vi "Main.vi"(11 "Module Admin":refnum<class "Delacor_lib_QMH_Module Admin.lvclass">) -> ()   [LabVIEW 2020, in "Peek Window.lvlib"]
doc: "This template is based off of the Queued Message Handler design pattern and the Queued Message Handler project template that ships with LabVIEW.\n\nThe main difference is that the queue is private to this module and communication between modules is performed via Broadcast and Request events.\n\nRequest events are wrapped in public API methods and are handled in the Event Handling Loop (EHL) of this VI. Any module can register for Broadcast events sent by this module. The EHL generates messages based on user interface actions.\n\nThe Message Handling Loop (MHL) processes messages generated by the EHL, or by other messages. The messages are string values, so new messages can be added easily to the Message Cases case structure in the MHL. Each message cluster can also provide an optional value for Message Data, which is a variant that can be converted to whatever message-specific data is required.\n_____\nBased on Delacor QMH Project Template 5.0.0.82."
uses:
  Peek Window.lvlib
  <vilib>/Delacor/Delacor QMH/Libraries/Module Admin_class/Delacor_lib_QMH_Module Admin.lvclass
  MHL Data Cluster.ctl
  VI Types/Standard VI Type/Standard VI Type.lvclass
  EHL Data Cluster.ctl
  <vilib>/Delacor/Delacor QMH/Libraries/Message Queue_class/Delacor_lib_QMH_Message Queue.lvclass/Delacor_lib_QMH_Message Queue.ctl
  Stop Argument--cluster.ctl
  Open Diagram Argument--cluster.ctl
  Invalid Selection Argument--cluster.ctl
  VI Types/Standard VI Type/Standard VI Type.lvclass/Standard VI Type.ctl
  Scroll Data.ctl
  <vilib>/Utility/traverseref.llb/TRef TravTarget.ctl
  <vilib>/Delacor/Delacor QMH/Libraries/Module Admin_class/Delacor_lib_QMH_Module Admin.lvclass/Delacor_lib_QMH_Module Admin.ctl
  <vilib>/Delacor/Delacor QMH/Libraries/Message Queue_class/Delacor_lib_QMH_Enqueue Message (Single).vi
  VI Types/Standard VI Type/Read VI Refnum.vi
  VI Types/Standard VI Type/Read Full Qualified Name.vi
  <vilib>/Delacor/Delacor QMH/Libraries/Module Admin_class/Delacor_lib_QMH_Get External Launch.vi
  <vilib>/Utility/error.llb/Error Cluster From Error Code.vi
  <vilib>/ErrorRing/Error Ring.xnode
  <vilib>/Delacor/Delacor QMH/Libraries/Message Queue_class/Delacor_lib_QMH_Message Queue.lvclass
  <vilib>/Utility/miscctls.llb/LVPoint32TypeDef.ctl
panel:
  in  "File Open":bool
  in  "Previous":bool
  in  "Peek Stack":string(tree)
  out "Application":string
  in  "Simulate MHL Error":bool
  in  "Simulate EHL Error":bool
  out "error out":errorcluster
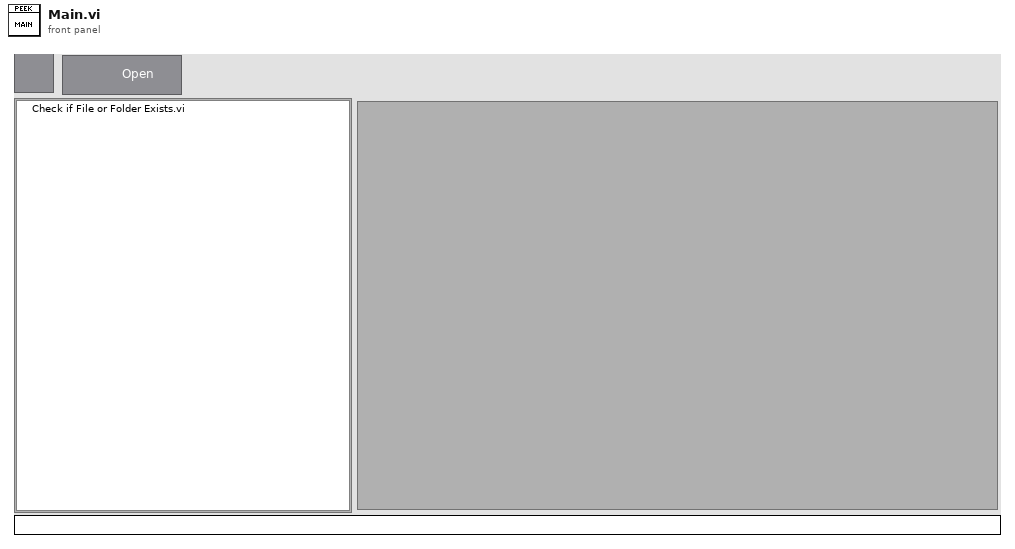
[diagram p1: front panel]
types:
  T1 = typedef "Peek Window.lvlib/EHL Data Cluster.ctl" = cluster{"VI Inserted":string, "Top VI":refnum<class "Standard VI Type.lvclass">}
  T2 = typedef "Peek Window.lvlib/MHL Data Cluster.ctl" = cluster{"PeekVI Reference":refnum<vi>, "SubPanel":refnum<vi>, "Peek Stack Tree Ref":refnum<vi>, "Open Button Ref":refnum<vi>, "Top VI":refnum<class "Standard VI Type.lvclass">, "Active VI":refnum<class "Standard VI Type.lvclass">, "Stack":refnum<class "Standard VI Type.lvclass">[], "Last FP State":enum32{"Invalid", "Standard", "Closed", "Hidden", "Minimized", "Maximized"}}
  T3 = typedef "Peek Window.lvlib/Request Events--cluster.ctl" = cluster{"Stop Module":refnum<user-event>, "Show Panel":refnum<user-event>, "Hide Panel":refnum<user-event>, "Get Module Execution Status":refnum<user-event>, "Show Diagram":refnum<user-event>, "Open Diagram":refnum<user-event>, "Invalid Selection":refnum<user-event>}
  T4 = enum32{"invalid lock state", "Not Locked", "Locked (No Password)", "Password-protected"}
  T5 = typedef "Peek Window.lvlib/Stop Argument--cluster.ctl" = cluster{"Origin":string, "Exit via Stop Module Req?":bool, "Wait for Module to stop?":bool}
  T6 = typedef "Peek Window.lvlib/Open Diagram Argument--cluster.ctl" = cluster{"VI Type":refnum<class "Standard VI Type.lvclass">}
  T7 = typedef "Peek Window.lvlib/Invalid Selection Argument--cluster.ctl" = cluster{"Active VI":string}
  T8 = enum32{"Invalid", "Standard", "Closed", "Hidden", "Minimized", "Maximized"}
  T9 = typedef "Peek Window.lvlib/Scroll Data.ctl" = cluster{"Coords":T10, "Delta":i32, "PlatMods":cluster{"Shift":bool, "Ctrl":bool, "Alt":bool, "Cmd":bool, "Opt":bool}}
  T10 = typedef "LVPoint32TypeDef.ctl" = cluster{"Horizontal":i32, "Vertical":i32}
  T11 = typedef "TRef TravTarget.ctl" = enum16{"FP", "BD", "Other"}
  T12 = cluster{"Shift":bool, "Ctrl":bool, "Alt":bool, "Cmd":bool, "Opt":bool}
  T13 = cluster{"Coords":T10, "Delta":i32, "PlatMods":cluster{"Shift":bool, "Ctrl":bool, "Alt":bool, "Cmd":bool, "Opt":bool}}
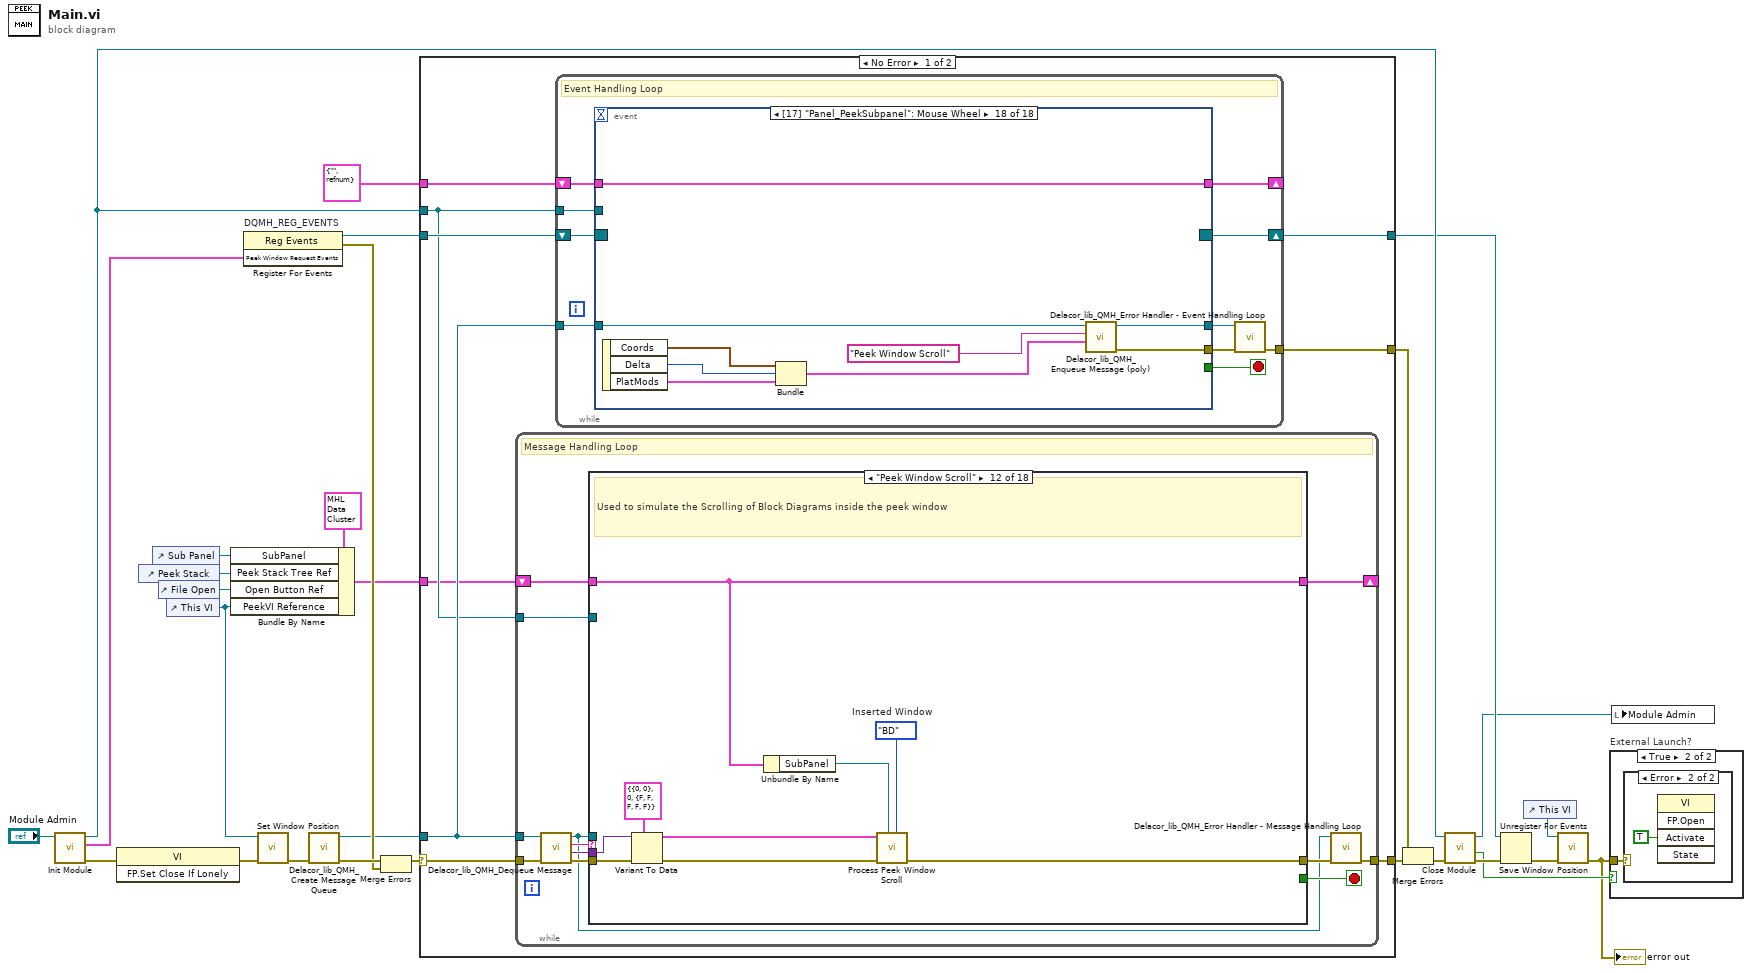
[diagram p0: block diagram]
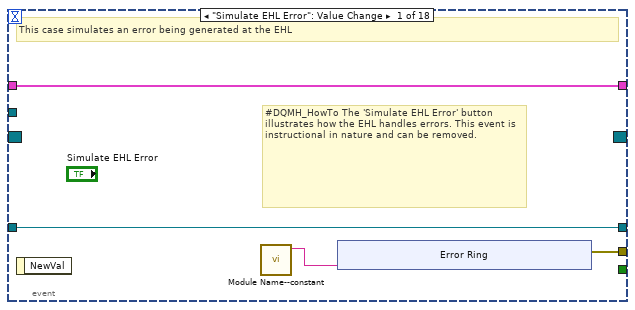
[diagram p2: hidden frame]
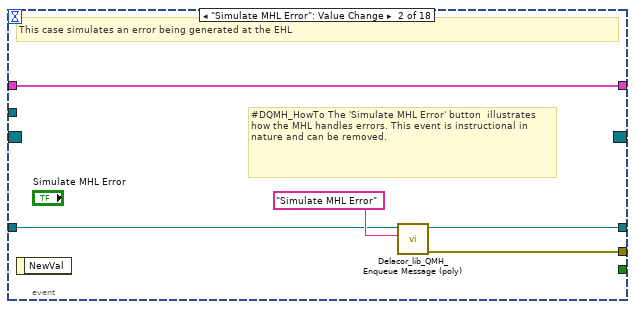
[diagram p3: hidden frame]
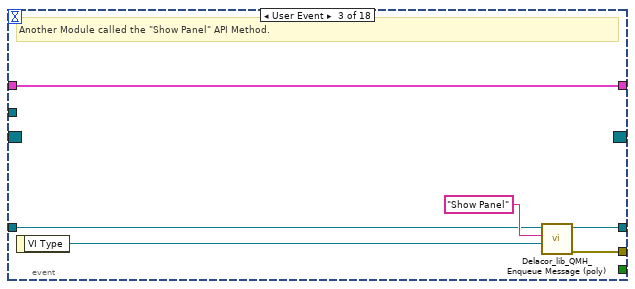
[diagram p4: hidden frame]
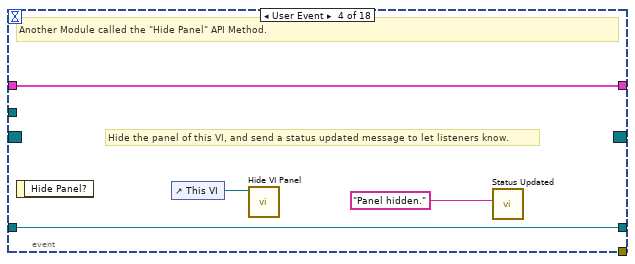
[diagram p5: hidden frame]
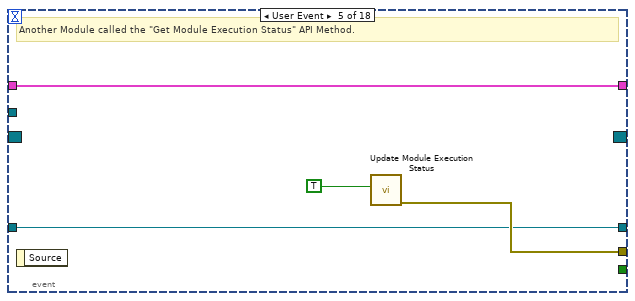
[diagram p6: hidden frame]
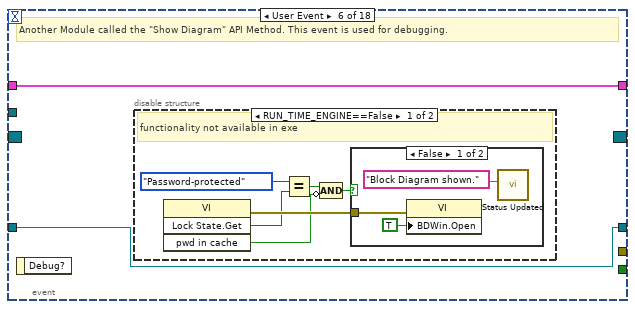
[diagram p7: hidden frame]
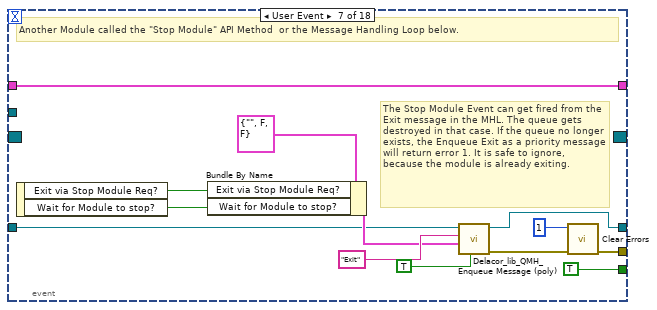
[diagram p10: hidden frame]
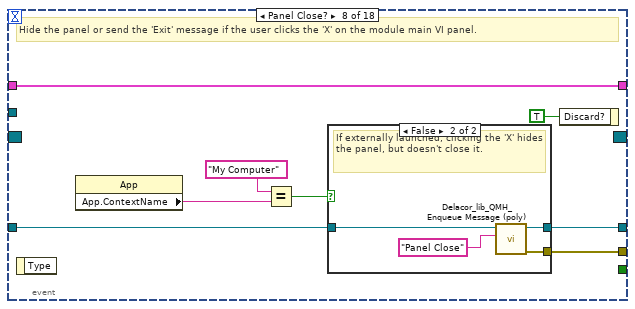
[diagram p11: hidden frame]
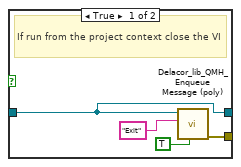
[diagram p12: hidden frame]
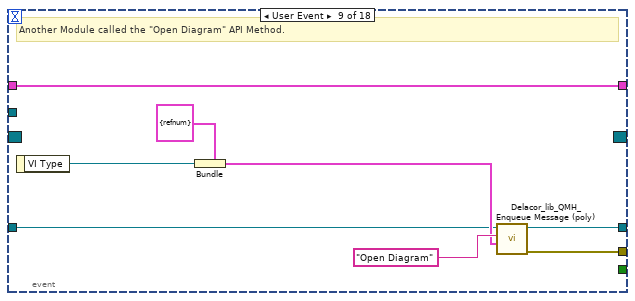
[diagram p13: hidden frame]
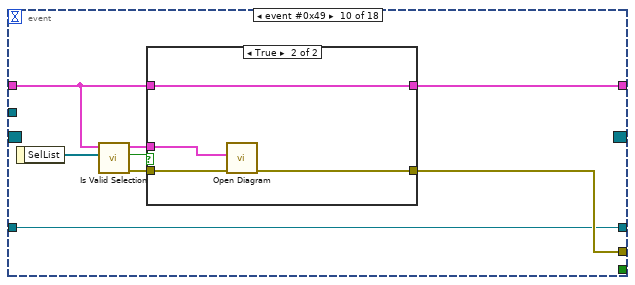
[diagram p14: hidden frame]
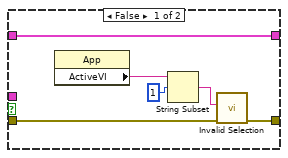
[diagram p15: hidden frame]
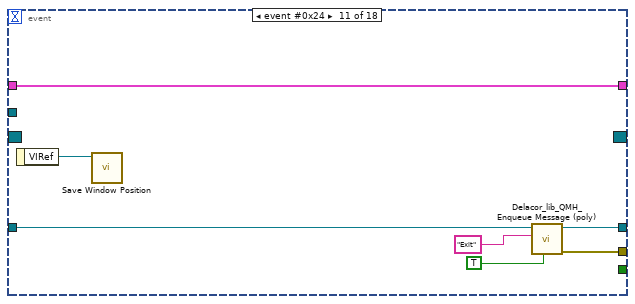
[diagram p16: hidden frame]
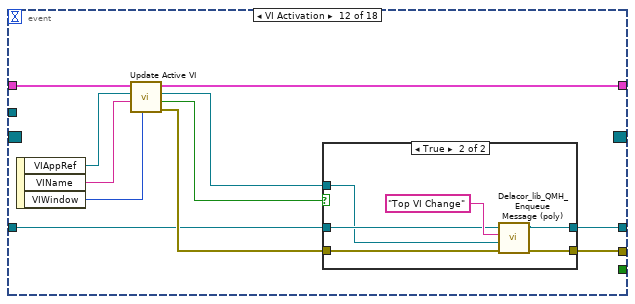
[diagram p17: hidden frame]
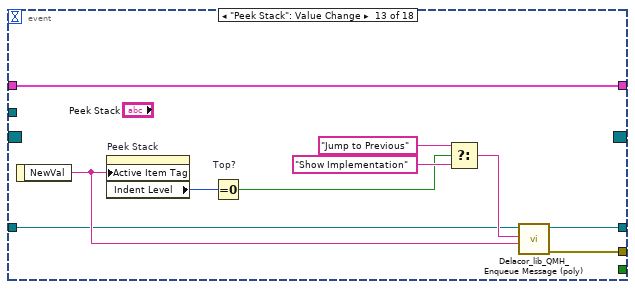
[diagram p19: hidden frame]
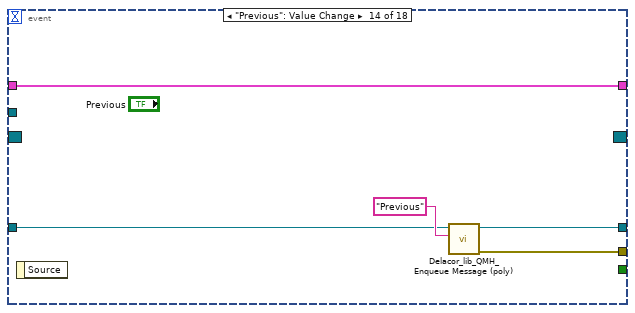
[diagram p20: hidden frame]
diagram:
  n1 = call "Init Module.vi"("Singleton Module Admin in"="Module Admin") -> ("error out"=w9:errorcluster, "Peek Window Request Events"=w18:T3, "Singleton Module Admin out"=w21:refnum<class "Delacor_lib_QMH_Module Admin.lvclass">)  [unwired: 8 in]
  n2 = invoke class="VI" method="FP.Set Close If Lonely"(error in=w9) -> (error out=w7:errorcluster)  [unwired: 2 in, 2 out]
  n3 = control-ref of="Peek Stack"() -> (w8:refnum<vi>)
  n4 = control-ref of="Sub Panel"() -> (w11:refnum<vi>)
  n5 = control-ref of="File Open"() -> (w1:refnum<vi>)
  n6 = control-ref of="This VI"() -> (w5:refnum<vi>)
  n7 = Bundle By Name(cluster=T2 {"PeekVI Reference"=refnum, "SubPanel"=refnum, "Peek Stack Tree Ref"=refnum, "Open Button Ref"=refnum, "Top VI"=refnum, "Active VI"=refnum, "Stack"=[], "Last FP State"=enum."Standard"} ("Data Cluster"), "SubPanel"=w11, "Peek Stack Tree Ref"=w8, "Open Button Ref"=w1, "PeekVI Reference"=w5) -> (w12:T2)
  n8 = register-events "DQMH_REG_EVENTS"(w18) -> (reference out=w19:refnum<event-registration>, error out=w22:errorcluster)  [unwired: 2 in]
  n9 = call "Set Window Position.vi"("error in"=w7, "VI Reference"=w5) -> ("error out"=w6:errorcluster)  [unwired: 9 in]
  n10 = call <vilib>:"Delacor_lib_QMH_Create Message Queue.vi"("error in"=w6) -> ("error out"=w24:errorcluster, "Message Queue"=w17:refnum<class "Delacor_lib_QMH_Message Queue.lvclass">)  [unwired: 9 in]
  n11 = Merge Errors(w24, w22) -> (w23:errorcluster)
  n12 = case shown="No Error" w23 {
    selector: w23 -> [w35 w498]
    tunnel: [w37 w497] -> w28
    tunnel: [w34 w503] -> w20
    tunnel: w19 -> [w33 w503]
    tunnel: w17 -> [w32 w496]
    tunnel: [w36 _] -> w26
    tunnel: w21 -> [w31 w499]
    tunnel: w12 -> [w30 _]
    tunnel: T1 {"VI Inserted"="", "Top VI"=refnum} ("Data") -> [w29 _]
    frame No Error {
      n13 = while {
        tunnel: w32 -> [w222]
        shift-right: [w219] -> _
        shift-left: w30 -> [w226]
        tunnel: w35 -> [w229]
        tunnel: [w227] -> w37
        tunnel: w31 -> [w220]
        stop <- w225 stop-if-true
        # "Message Handling Loop"
        n14 = call-dynamic "Delacor_lib_QMH_Dequeue Message.vi"("error in"=w229, "Message Queue in"=w222) -> ("error out"=w228:errorcluster, "Message Data"=w223:variant, "Message"=w224:string, "Message Queue out"=w221:refnum<class "Delacor_lib_QMH_Message Queue.lvclass">)  [unwired: 6 in]
        n15 = case "DQMH_MESSAGE_CASES" shown="\"Peek Window Scroll\"" w224 {
          selector: w224 -> [_ _ _ _ _ _ _ _ _ _ _ _ _ _ _ _ _ w483]
          tunnel: w221 -> [_ _ _ _ _ _ _ _ _ _ _ _ _ _ _ w453 w475 _]
          tunnel: w228 -> [w241 w243 w250 w265 w299 w316 w342 w354 w367 w384 w412 w432 w435 w437 w442 w460 w481 w485]
          tunnel: [w231 w243 w245 w262 w297 w319 w336 w351 w368 w383 w404 w427 w434 w437 w441 w456 w478 w486] -> w230
          tunnel: w226 -> [w235 w242 w246 w259 w293 w317 w333 w357 w363 w388 w400 w426 w433 w436 w439 w455 w474 w484]
          tunnel: [w232 w242 w247 w260 w296 w318 w334 w356 w361 w387 w399 w426 w433 w436 w439 w455 w474 w484] -> w219
          tunnel: [_ _ _ _ _ _ _ _ _ _ _ _ _ _ _ _ w473 _] -> w225
          tunnel: w223 -> [_ _ w249 w264 w298 _ w340 _ w365 _ w411 w430 _ _ _ w454 w472 _]
          tunnel: w220 -> [w238 _ _ _ _ _ _ _ _ _ _ _ _ _ _ w452 w467 _]
          frame "Initialize" {
            # "Initialize - Any operation that needs to be done before the module can receive messages. Synchronize Caller Events.vi will inform Start Module.vi that the module has launched and is ready to receive messages. Module Did Init.vi will broadcast that the module initialized."
            n16 = call "Synchronize Caller Events.vi"("error in (no error)"=w241, "Singleton Module Admin in"=w238) -> ("error out"=w240:errorcluster)  [unwired: 8 in, 1 out]
            n17 = call "Module Name--constant.vi"() -> ("Module Name"=w239:string)  [unwired: 11 in]
            n18 = property on="Property Node" class="VI"("Front Panel.Title"=w239) -> (reference out=w233:refnum<vi>)  [unwired: 2 in, 1 out]
            n19 = call "Initialize Tree.vi"("Module Data"=w235) -> ("Module Data"=w232:T2)  [unwired: 9 in, 1 out]
            n20 = call "Module Name--constant.vi"() -> ("Module Name"=w236:string)  [unwired: 11 in]
            n21 = property on="Property Node" class="VI"(reference=w233, "FP.State"=T8."Standard" ("Front Panel Window:State")) -> ()  [unwired: 1 in, 2 out]
            n22 = call "Module Did Init.vi"("error in (no error)"=w240, "Initialized?"=TRUE, "Origin"=w236) -> ("error out"=w231:errorcluster)  [unwired: 8 in]
          }
          frame "--- Module Specific ---" {
            # "Separator -- The following cases handle messages specific to this Module."
          }
          frame "Top VI Change" {
            w248 = refnum<class "Standard VI Type.lvclass"> refnum  # Top VI
            # "Open BD of selected SubVI"
            n23 = Variant To Data(error in=w250, type=w248, Variant=w249) -> (data=w244:refnum<class "Standard VI Type.lvclass">, error out=w245:errorcluster)
            n24 = Bundle By Name(cluster=w246, "Top VI"=w244) -> (w247:T2)
          }
          frame "Open Diagram" {
            # "Open BD of selected SubVI"
            n25 = Variant To Data(error in=w265, type=T6 {"VI Type"=refnum} ("Open Diagram Argument"), Variant=w264) -> (data=w252:T6, error out=w255:errorcluster)
            n26 = Unbundle By Name(w252) -> ("VI Type"=w251:refnum<class "Standard VI Type.lvclass">)
            n27 = Unbundle By Name(w259) -> ("Stack"=w258:refnum<class "Standard VI Type.lvclass">[])
            n28 = Search 1D Array(1D array=w258, element=w251) -> (index of element=w261:i32)  [unwired: 1 in]
            n29 = call-dynamic "Check if Open or Locked.vi"("error in (no error)"=w255, "Standard VI Type in"=w251) -> ("error out"=w254:errorcluster, "Openable?"=w253:bool)  [unwired: 8 in]
            n30 = Less Than 0?(x=w261) -> (x < 0?=w257:bool)
            n31 = And(x=w257, y=w253) -> (x .and. y?=w256:bool)
            n32 = case shown="True" w256 {
              tunnel: [w269 w283] -> w262
              tunnel: w254 -> [w268 w275]
              tunnel: [w267 w277] -> w260
              tunnel: w259 -> [w267 w280]
              tunnel: w251 -> [w270 w271]
              frame False {
                n33 = Unbundle By Name(w267) -> ("SubPanel"=w266:refnum<vi>)
                n34 = call-dynamic "Display Unopenable Message.vi"("error in (no error)"=w268, "SubPanel"=w266, "Standard VI Type in"=w270) -> ("error out"=w269:errorcluster)  [unwired: 7 in, 1 out]
              }
              frame True {
                n35 = Bundle By Name(cluster=w280, "Active VI"=w271) -> (w279:T2)
                n36 = call "Get Application Instance Name.vi"("VI Type"=w271) -> ("Name"=→"Application":string)  [unwired: 10 in]
                n37 = Bundle By Name(cluster=T6 {"VI Type"=refnum} ("Open Diagram Argument"), "VI Type"=w271) -> (w273:T6)
                n38 = call "Update Call Chain.vi"("error in (no error)"=w275, "Data Cluster in"=w279) -> ("error out"=w284:errorcluster, "Data Cluster out"=w282:T2)  [unwired: 8 in]
                n39 = call "Add to Tree.vi"("error in"=w284, "Data in"=w282) -> ("error out"=w276:errorcluster, "Data out"=w278:T2)  [unwired: 8 in]
                n40 = call "Insert Into Subpanel.vi"("error in (no error)"=w276, "Data in"=w278) -> ("error out"=w274:errorcluster, "Data out"=w277:T2)  [unwired: 8 in]
                n41 = call "Show Panel.vi"("error in (no error)"=w274, "Open Diagram Argument"=w273) -> ("error out"=w283:errorcluster)  [unwired: 9 in]
              }
            }
          }
          frame "Show Implementation" {
            # "This event is returned by the Choose Implementation popup for dynamic dispatch VIs.  It causes the implementation to be shown in the subpanel."
            n42 = Variant To Data(error in=w299, type="", Variant=w298) -> (data=w292:string, error out=w290:errorcluster)
            n43 = call "Lookup Implementor.vi"("error in (no error)"=w290, "Implementor ID"=w292, "Data in"=w293) -> ("error out"=w287:errorcluster, "Found?"=w291:bool, "Data out"=w289:T2)  [unwired: 6 in]
            n44 = Unbundle By Name(w289) -> ("Active VI"=w288:refnum<class "Standard VI Type.lvclass">)
            n45 = call-dynamic "Check if Open or Locked.vi"("error in (no error)"=w287, "Standard VI Type in"=w288) -> ("error out"=w286:errorcluster, "Openable?"=w285:bool)  [unwired: 8 in]
            n46 = Compound Arithmetic op=AND "Found\nAND\nOpenable"(w291, w285) -> (w295:bool)
            n47 = case shown="True" w295 {
              tunnel: [w301 w313] -> w297
              tunnel: w286 -> [w300 w307]
              tunnel: [w303 w312] -> w296
              tunnel: w289 -> [w303 w309]
              frame False {
                n48 = Unbundle By Name(w303) -> ("Active VI"=w302:refnum<class "Standard VI Type.lvclass">, "SubPanel"=w304:refnum<vi>)
                n49 = call-dynamic "Display Unopenable Message.vi"("error in (no error)"=w300, "SubPanel"=w304, "Standard VI Type in"=w302) -> ("error out"=w301:errorcluster)  [unwired: 7 in, 1 out]
              }
              frame True {
                n50 = call "Replace Item in Peek Stack.vi"("error in (no error)"=w307, "Data Cluster in"=w309) -> ("error out"=w306:errorcluster, "Active VI Previous State"=w305:refnum<class "Standard VI Type.lvclass">, "Data Cluster out"=w308:T2)  [unwired: 7 in]
                n51 = call "Replace Item in Tree.vi"("error in"=w306, "Active VI Previous State"=w305, "Module Data"=w308) -> ("error out"=w311:errorcluster, "Module Data"=w310:T2)  [unwired: 7 in]
                n52 = call "Insert Into Subpanel.vi"("error in (no error)"=w311, "Data in"=w310) -> ("error out"=w313:errorcluster, "Data out"=w312:T2)  [unwired: 8 in]
              }
            }
          }
          frame "Previous" {
            # "Open BD of previous SubVI"
            n53 = Unbundle By Name(w317) -> ("Stack"=w314:refnum<class "Standard VI Type.lvclass">[])
            n54 = Array Size(array=w314) -> (size(s)=w315:i32)
            n55 = case shown="2.." w315 {
              tunnel: [w322 w329] -> w319
              tunnel: [w320 w332] -> w318
              tunnel: w317 -> [w328 w331]
              tunnel: w316 -> [w327 w330]
              frame 2.. {
                # "More than 1 item in Peek Stack"
                n56 = call "Remove Last Item from Peek Stack.vi"("error in (no error)"=w327, "Data Cluster in"=w328) -> ("error out"=w324:errorcluster, "Removed VI"=w326:refnum<class "Standard VI Type.lvclass">, "Data Cluster out"=w325:T2)  [unwired: 7 in]
                n57 = call "Delete Last Item.vi"("error in (no error)"=w324, "Removed VI"=w326, "Data Cluster"=w325) -> ("error out"=w323:errorcluster, "Module Data"=w321:T2)  [unwired: 7 in]
                n58 = call "Insert Into Subpanel.vi"("error in (no error)"=w323, "Data in"=w321) -> ("error out"=w322:errorcluster, "Data out"=w320:T2)  [unwired: 8 in]
              }
              frame ..1 {
                # "1 Item in Peek Stack"
                n59 = call "Highlight Top SubVI.vi"("error in (no error)"=w330, "Data in"=w331) -> ("error out"=w329:errorcluster, "Data out"=w332:T2)  [unwired: 8 in]
              }
            }
          }
          frame "Jump to Previous" {
            n60 = Variant To Data(error in=w342, type="", Variant=w340) -> (data=w338:string, error out=w341:errorcluster)
            n61 = call "Jump Back.vi"("error in"=w341, "VI Name"=w338, "Data in"=w333) -> ("error out"=w337:errorcluster, "Data out"=w335:T2)  [unwired: 7 in]
            n62 = call "Insert Into Subpanel.vi"("error in (no error)"=w337, "Data in"=w335) -> ("error out"=w336:errorcluster, "Data out"=w334:T2)  [unwired: 8 in]
          }
          frame "File Open" {
            w347 = refnum<class "Standard VI Type.lvclass">[] []  # Reset Stack
            # "Open VI in Current Window"
            n63 = Unbundle By Name(w357) -> ("Stack"=w355:refnum<class "Standard VI Type.lvclass">[], "SubPanel"=w353:refnum<vi>)
            n64 = invoke class="SubPnl" method="Remove VI"(reference=w353, error in=w354) -> (error out=w350:errorcluster)  [unwired: 1 in, 2 out]
            n65 = Delete From Array(array=w355) -> (deleted portion=w346:refnum<class "Standard VI Type.lvclass">)  [unwired: 2 in, 1 out]
            n66 = property class="VI"(error in=w350, "FP.State"=T8."Hidden" ("Front Panel Window:State")) -> (error out=w344:errorcluster)  [unwired: 1 in, 1 out]
            n67 = property class="Standard VI Type"(reference=w346, error in=w344) -> (error out=w343:errorcluster, "Accessors:VI Refnum"=w345:refnum<vi>)  [unwired: 1 out]
            n68 = Bundle By Name(cluster=w357, "Stack"=w347) -> (w356:T2)
            n69 = property class="VI"(reference=w345, error in=w343, "BDWin.Open"=TRUE ("Block Diagram Window:Open"), "FP.State"=T8."Minimized" ("Front Panel Window:State")) -> (error out=w351:errorcluster)  [unwired: 1 out]
          }
          frame "Show Panel" {
            w360 = refnum<class "Standard VI Type.lvclass"> refnum  # Active VI
            n70 = Variant To Data(error in=w367, type=w360, Variant=w365) -> (data=w359:refnum<class "Standard VI Type.lvclass">, error out=w366:errorcluster)
            n71 = Bundle By Name(cluster=w363, "Active VI"=w359) -> (w362:T2)
            n72 = Unbundle By Name(w362) -> ("Stack"=w358:refnum<class "Standard VI Type.lvclass">[])
            n73 = Empty Array?(array=w358) -> (empty?=w364:bool)
            n74 = case shown="False" w364 {
              tunnel: [w374 w379] -> w368
              tunnel: w366 -> [w374 w379]
              tunnel: w362 -> [w370 w378]
              tunnel: [w369 w378] -> w361
              frame False {
                # "Call Chain not empty"
                n75 = property class="VI"() -> ("FP.State"=w373:T8)  [unwired: 2 in, 2 out]
                n76 = Equal?(x=w373, y=T8."Hidden") -> (x = y?=w371:bool)
                n77 = case shown="True" w371 {
                  tunnel: w370 -> [w375 w377]
                  tunnel: [w375 w377] -> w369
                  frame False {
                  }
                  frame True {
                    n78 = Unbundle By Name(w377) -> ("Last FP State"=w376:T8)
                    n79 = property class="VI"("FP.State"=w376) -> ()  [unwired: 2 in, 2 out]
                  }
                }
              }
              frame True {
                # "Nothing in Call Chain"
              }
            }
          }
          frame "Panel Close" {
            # "User Closed VI-Peek"
            n80 = property class="VI"(error in=w384) -> (error out=w385:errorcluster, "FP.State"=w382:T8)  [unwired: 1 in, 1 out]
            n81 = Equal?(x=T8."Hidden", y=w382) -> (x = y?=w380:bool)
            n82 = case "Race condition from user clicking panel close before this message executes" shown="True" w380 {
              tunnel: w388 -> [w390 w396]
              tunnel: [w392 w395] -> w387
              tunnel: w382 -> [_ w393]
              frame True {
                n83 = Unbundle By Name(w390) -> ("Last FP State"=w389:T8)
                n84 = Bundle By Name(cluster=w390, "Stack"=refnum<class "Standard VI Type.lvclass">[] [], "Last FP State"=w389) -> (w392:T2)
              }
              frame False {
                n85 = Bundle By Name(cluster=w396, "Stack"=refnum<class "Standard VI Type.lvclass">[] [], "Last FP State"=w393) -> (w395:T2)
              }
            }
            n86 = control-ref of="This VI"() -> (w386:refnum<vi>)
            n87 = call "Hide VI Panel.vi"("error in (no error)"=w385, "VI"=w386) -> ("error out"=w383:errorcluster)  [unwired: 9 in]
          }
          frame "Invalid Selection" {
            n88 = Unbundle By Name(w400) -> ("Stack"=w398:refnum<class "Standard VI Type.lvclass">[])
            n89 = Variant To Data(error in=w412, type=T7 {"Active VI"=""} ("Invalid Selection Argument"), Variant=w411) -> (data=w409:T7, error out=w405:errorcluster)
            n90 = for {
              tunnel: w398 -> [w414] mode=indexing
              tunnel: [w413] -> w397 mode=indexing
              n91 = property class="Standard VI Type"(reference=w414) -> ("Accessors:Full Qualified Name"=w413:string)  [unwired: 1 in, 2 out]
            }
            n92 = Unbundle By Name(w409) -> ("Active VI"=w406:string)
            n93 = property class="VI"() -> ("Name"=w408:string)  [unwired: 2 in, 2 out]
            n94 = Build Array (concatenate)(w397, w408, "VI Hierarchy") -> (w407:string[])
            n95 = Search 1D Array(1D array=w407, element=w406) -> (index of element=w403:i32)  [unwired: 1 in]
            n96 = Less Than 0?(x=w403) -> (x < 0?=w402:bool)
            n97 = case shown="True" w402 {
              tunnel: w405 -> [w416 w419]
              tunnel: [w416 w418] -> w404
              tunnel: w400 -> [w415 w421]
              tunnel: [w415 w422] -> w399
              frame False {
              }
              frame True {
                w417 = refnum<class "Standard VI Type.lvclass">[] []  # Stack
                n98 = Unbundle By Name(w421) -> ("SubPanel"=w420:refnum<vi>)
                n99 = invoke class="SubPnl" method="Remove VI"(reference=w420, error in=w419) -> (error out=w418:errorcluster)  [unwired: 1 in, 2 out]
                n100 = property class="VI"("FP.State"=T8."Hidden" ("Front Panel Window:State")) -> ()  [unwired: 2 in, 2 out]
                n101 = Bundle By Name(cluster=w421, "Stack"=w417) -> (w422:T2)
              }
            }
          }
          frame "Peek Window Scroll" {
            w424 = TRef_TravTarget."BD"  # Inserted Window
            # "Used to simulate the Scrolling of Block Diagrams inside the peek window"
            n102 = Variant To Data(error in=w432, type=T9 {"Coords"={"Horizontal"=0, "Vertical"=0}, "Delta"=0, "PlatMods"={"Shift"=FALSE, "Ctrl"=FALSE, "Alt"=FALSE, "Cmd"=FALSE, "Opt"=FALSE}} ("Process Peek Window Scroll Argument"), Variant=w430) -> (data=w428:T9, error out=w431:errorcluster)
            n103 = Unbundle By Name(w426) -> ("SubPanel"=w425:refnum<vi>)
            n104 = call "Process Peek Window Scroll.vi"("Inserted Window"=w424, "SubPanel"=w425, "error in (no error)"=w431, "Process Peek Window Scroll Argument"=w428) -> ("error out"=w427:errorcluster)  [unwired: 5 in]
          }
          frame "---Copy This Frame---" {
            # "Duplicate this frame when creating new messages.  Change this comment in the duplicated frame to describe this message."
            n105 = Merge Errors(w435) -> (w434:errorcluster)
          }
          frame "--- Exit and Error Handling---" {
            # "Separator - The following cases handle errors and exit messages."
          }
          frame "Simulate MHL Error" {
            # "#DQMH_HowTo The 'Simulate MHL Error' button  illustrates how the MHL handles errors. This event is instructional in nature and can be removed."
            # "Simulate an error occurring at the MHL"
            n106 = call "Module Name--constant.vi"() -> ("Module Name"=w438:string)  [unwired: 11 in]
            n107 = xnode "Error Ring"("parameter 0"=w438) -> ("error out"=w440:errorcluster)
            n108 = Merge Errors(w442, w440) -> (w441:errorcluster)
          }
          frame "Error" {
            # "#CodeRecommended - If you ever change the name of this \"Error\" message, you'll need to update the name in the Check Loop Error.vi as well."
            # "#CodeRecommended - If the module is running in standalone mode (External Launch = FALSE), this code will pop up an error dialog and call the 'Exit' message if an error occurs. Add more fine-grained error handling here."
            # "Error - Check the error message data and respond accordingly. This message is sent by the \"Error Handler\" VIs at the end of each loop in this application."
            n109 = property on="Property Node" class="Module Admin"(reference=w452) -> ("Accessors:External Launch"=w451:bool)  [unwired: 1 in, 2 out]
            n110 = Variant To Data(error in=w460, type=errorcluster {"status"=FALSE, "code"=0, "source"=""} ("error constant"), Variant=w454) -> (data=w461:errorcluster, error out=w458:errorcluster)
            n111 = call "Module Name--constant.vi"() -> ("Module Name"=w450:string)  [unwired: 11 in]
            n112 = call "Error Reported.vi"("Additional Information"=w450, "Error"=w461) -> ()  [unwired: 9 in, 1 out]
            n113 = case shown="False" w451 {
              tunnel: [w466 _] -> w457
              tunnel: w453 -> [w464 _]
              tunnel: w461 -> [w465 _]
              frame False {
                # "If the module is running standalone, then pop up an error dialog and call the \"Exit\" message."
                n114 = call <vilib>:"Simple Error Handler.vi"("error in (no error)"=w465) -> ()  [unwired: 4 in, 5 out]
                n115 = call-poly <vilib>:"Delacor_lib_QMH_Enqueue Message (poly).vi"("Priority Message? (F)"=TRUE, "Message"="Exit", "Message Queue in"=w464) -> ("error out"=w466:errorcluster)  [unwired: 7 in, 1 out]
              }
              frame True {
                # "If the module was launched externally, calling the Error Reported broadcast VI is the only action performed by the \"Error\" message. The module's caller can then process the error appropriately."
              }
            }
            n116 = Merge Errors(w458, w457) -> (w456:errorcluster)
            n117 = local write "error out"(w456) -> ()
          }
          frame "Exit" {
            w471 = 91  # 91: not all Exit messages will have an argument
            w473 = TRUE  # Stop the VI
            # "Release the message queue reference"
            # "#CodeNeeded - Add any required cleanup code here"
            # "Exit - Exit the application."
            n118 = Variant To Data(error in=w481, type=T5 {"Origin"="", "Exit via Stop Module Req?"=FALSE, "Wait for Module to stop?"=FALSE} ("Stop Argument"), Variant=w472) -> (data=w469:T5, error out=w477:errorcluster)
            n119 = call <vilib>:"Clear Errors.vi"("error in (no error)"=w477, "specific error code to clear (0: all)"=w471) -> ("error out"=w480:errorcluster)  [unwired: 4 in, 1 out]
            n120 = control-ref of="This VI"() -> (w468:refnum<vi>)
            n121 = call-dynamic "Delacor_lib_QMH_Release Message Queue.vi"("error in"=w480, "Message Queue"=w475) -> ("error out"=w479:errorcluster)  [unwired: 9 in]
            n122 = call "Handle Exit.vi"("Stop Argument"=w469, "Admin in"=w467, "VI reference"=w468) -> ("error out"=w476:errorcluster)  [unwired: 7 in, 1 out]
            n123 = Merge Errors(w479, w476) -> (w478:errorcluster)
          }
          frame Default {
            # "'Default' case only runs if there is a message that isn't defined in any of the other cases.  Output a programming error."
            n124 = call "Module Name--constant.vi"() -> ("Module Name"=w482:string)  [unwired: 11 in]
            n125 = xnode "Error Ring"("parameter 0"=w483, "parameter 1"=w482) -> ("error out"=w487:errorcluster)
            n126 = Merge Errors(w485, w487) -> (w486:errorcluster)
          }
        }
        n127 = call-dynamic "Delacor_lib_QMH_Error Handler - Message Handling Loop.vi"("error in"=w230, "Message Queue in"=w221) -> ("dup error in"=w227:errorcluster)  [unwired: 8 in, 1 out]
      }
      n128 = while {
        tunnel: w32 -> [w39]
        shift-right: [w44] -> w34
        shift-left: w33 -> [w45]
        tunnel: [w46] -> w36
        tunnel: w31 -> [w42]
        shift-right: [w40] -> _
        shift-left: w29 -> [w41]
        stop <- w43 stop-if-true
        # "Event Handling Loop"
        n129 = event "DQMH_EVENT_MAIN" shown="[17] \"Panel_PeekSubpanel\": Mouse Wheel" {
          selector: w45 -> [_ _ _ _ _ _ _ _ _ _ _ _ _ _ _ _ _ _]
          dyn-events: [_ _ _ _ _ _ _ _ _ _ _ _ _ _ _ _ _ _] -> w44
          timeout: _ -> [_ _ _ _ _ _ _ _ _ _ _ _ _ _ _ _ _ _]
          tunnel: [_ _ _ _ _ _ TRUE ("Discard?") _ _ _ _ _ _ _ _ _ _ _] -> w43
          tunnel: w39 -> [w48 w59 w64 w70 w74 w78 w89 w102 w118 w126 w144 w151 w170 w181 w189 w197 w202 w212]
          tunnel: [w51 w63 w68 _ w77 _ w100 w109 w122 w131 w147 w156 w179 w184 w191 w200 w204 w210] -> w47
          tunnel: w42 -> [_ _ _ _ _ _ _ _ _ _ _ _ _ _ _ _ _ _]
          tunnel: w41 -> [w49 w61 w69 w71 w75 w79 w91 w107 w121 w128 w150 w158 w173 w182 w190 w201 w209 w218]
          tunnel: [w49 w61 w69 w71 w75 w79 w91 w107 w121 w127 w150 w161 w173 w182 w190 w201 w209 w218] -> w40
          tunnel: [w48 w60 w65 w70 w74 w78 w90 w103 w119 w126 w145 w152 w171 w180 w188 w198 w203 w211] -> w38
          event "Simulate EHL Error": Value Change {
            # "#DQMH_HowTo The 'Simulate EHL Error' button  illustrates how the EHL handles errors. This event is instructional in nature and can be removed."
            # "This case simulates an error being generated at the EHL"
            n130 = event-data() -> ()  [unwired: 1 in, 1 out]
            n131 = call "Module Name--constant.vi"() -> ("Module Name"=w50:string)  [unwired: 11 in]
            n132 = xnode "Error Ring"("parameter 0"=w50) -> ("error out"=w51:errorcluster)
          }
          event "Simulate MHL Error": Value Change {
            # "#DQMH_HowTo The 'Simulate MHL Error' button  illustrates how the MHL handles errors. This event is instructional in nature and can be removed."
            # "This case simulates an error being generated at the EHL"
            n133 = event-data() -> ()  [unwired: 1 in, 1 out]
            n134 = call-poly <vilib>:"Delacor_lib_QMH_Enqueue Message (poly).vi"("Message"="Simulate MHL Error", "Message Queue in"=w59) -> ("error out"=w63:errorcluster, "Message Queue out"=w60:refnum<class "Delacor_lib_QMH_Message Queue.lvclass">)  [unwired: 8 in]
          }
          event User Event {
            # "Another Module called the \"Show Panel\" API Method."
            n135 = event-data() -> ("VI Type"=w66:refnum<class "Standard VI Type.lvclass">)  [unwired: 1 in]
            n136 = call-poly <vilib>:"Delacor_lib_QMH_Enqueue Message (poly).vi"("Message Data"=w66, "Message"="Show Panel", "Message Queue in"=w64) -> ("error out"=w68:errorcluster, "Message Queue out"=w65:refnum<class "Delacor_lib_QMH_Message Queue.lvclass">)  [unwired: 7 in]
          }
          event User Event {
            # "Hide the panel of this VI, and send a status updated message to let listeners know."
            # "Another Module called the \"Hide Panel\" API Method."
            n137 = event-data() -> ()  [unwired: 1 in, 1 out]
            n138 = control-ref of="This VI"() -> (w73:refnum<vi>)
            n139 = call "Hide VI Panel.vi"("VI"=w73) -> ()  [unwired: 10 in, 1 out]
            n140 = call "Status Updated.vi"("Status"="Panel hidden." ("format string")) -> ()  [unwired: 10 in, 1 out]
          }
          event User Event {
            # "Another Module called the \"Get Module Execution Status\" API Method."
            n141 = event-data() -> ()  [unwired: 1 in, 1 out]
            n142 = call "Update Module Execution Status.vi"("Running?"=TRUE) -> ("error out"=w77:errorcluster)  [unwired: 10 in]
          }
          event User Event {
            # "Another Module called the \"Show Diagram\" API Method. This event is used for debugging."
            n143 = event-data() -> ()  [unwired: 1 in, 1 out]
            n144 = disable-structure shown="RUN_TIME_ENGINE==False" {
              frame condition #0 (active) {
                # "functionality not available in exe"
                n145 = invoke on="Invoke Node" class="VI" method="Lock State.Get"() -> (error out=w85:errorcluster, "Get Lock State"=w84:T4, "pwd in cache"=w81:bool)  [unwired: 4 in, 1 out]
                n146 = Equal?(x=T4."Password-protected", y=w84) -> (x = y?=w82:bool)
                n147 = Compound Arithmetic op=AND(w82, invert w81) -> (w80:bool)
                n148 = case shown="False" w80 {
                  tunnel: w85 -> [w88 _]
                  frame False {
                    n149 = property on="Property Node" class="VI"(error in=w88, "BDWin.Open"=TRUE ("Block Diagram Window:Open")) -> ()  [unwired: 1 in, 2 out]
                    n150 = call "Status Updated.vi"("Status"="Block Diagram shown." ("format string")) -> ()  [unwired: 10 in, 1 out]
                  }
                  frame True {
                    # "Password-protected VI, and the password is not in the cache. Do not show the diagram."
                  }
                }
              }
              frame condition #1 {
              }
            }
          }
          event User Event {
            # "The Stop Module Event can get fired from the Exit message in the MHL. The queue gets destroyed in that case. If the queue no longer exists, the Enqueue Exit as a priority message will return error 1. It is safe to ignore, because the module is already exiting."
            # "Another Module called the \"Stop Module\" API Method  or the Message Handling Loop below."
            n151 = event-data() -> ("Exit via Stop Module Req?"=w94:bool, "Wait for Module to stop?"=w93:bool)  [unwired: 1 in]
            n152 = Bundle By Name(cluster=T5 {"Origin"="", "Exit via Stop Module Req?"=FALSE, "Wait for Module to stop?"=FALSE} ("Stop Argument"), "Exit via Stop Module Req?"=w94, "Wait for Module to stop?"=w93) -> (w92:T5)
            n153 = call-poly <vilib>:"Delacor_lib_QMH_Enqueue Message (poly).vi"("Priority Message? (F)"=TRUE, "Message Data"=w92, "Message"="Exit", "Message Queue in"=w89) -> ("error out"=w101:errorcluster, "Message Queue out"=w90:refnum<class "Delacor_lib_QMH_Message Queue.lvclass">)  [unwired: 6 in]
            n154 = call <vilib>:"Clear Errors.vi"("error in (no error)"=w101, "specific error code to clear (0: all)"=1) -> ("error out"=w100:errorcluster)  [unwired: 4 in, 1 out]
          }
          event Panel Close? {
            # "Hide the panel or send the 'Exit' message if the user clicks the 'X' on the module main VI panel."
            n155 = event-data() -> ()  [unwired: 1 in, 1 out]
            n156 = property class="App"() -> ("App.ContextName"=w106:string)  [unwired: 2 in, 2 out]
            n157 = Equal?(x="My Computer", y=w106) -> (x = y?=w104:bool)
            n158 = case shown="False" w104 {
              tunnel: w102 -> [w112 w117]
              tunnel: [w113 w116] -> w109
              tunnel: [w112 w114] -> w103
              frame True {
                # "If run from the project context close the VI"
                n159 = call-poly <vilib>:"Delacor_lib_QMH_Enqueue Message (poly).vi"("Priority Message? (F)"=TRUE, "Message"="Exit", "Message Queue in"=w112) -> ("error out"=w113:errorcluster)  [unwired: 7 in, 1 out]
              }
              frame False {
                # "If externally launched, clicking the 'X' hides the panel, but doesn't close it."
                n160 = call-poly <vilib>:"Delacor_lib_QMH_Enqueue Message (poly).vi"("Message"="Panel Close", "Message Queue in"=w117) -> ("error out"=w116:errorcluster, "Message Queue out"=w114:refnum<class "Delacor_lib_QMH_Message Queue.lvclass">)  [unwired: 8 in]
              }
            }
            n161 = event-data ("Event Filter Node")("Discard?"=TRUE ("Discard the event, the MHL is responsible for closing and stopping this VI.")) -> ()  [unwired: 1 in, 1 out]
          }
          event User Event {
            # "Another Module called the \"Open Diagram\" API Method."
            n162 = event-data() -> ("VI Type"=w120:refnum<class "Standard VI Type.lvclass">)  [unwired: 1 in]
            n163 = Bundle(cluster=T6 {"VI Type"=refnum} ("Open Diagram Argument"), "VI Type"=w120) -> (w123:T6)
            n164 = call-poly <vilib>:"Delacor_lib_QMH_Enqueue Message (poly).vi"("Message Data"=w123, "Message"="Open Diagram", "Message Queue in"=w118) -> ("error out"=w122:errorcluster, "Message Queue out"=w119:refnum<class "Delacor_lib_QMH_Message Queue.lvclass">)  [unwired: 7 in]
          }
          event event #0x49 {
            n165 = event-data() -> ("SelList"=w130:refnum<vi>[])  [unwired: 1 in]
            n166 = call "Is Valid Selection"("SelList"=w130, "Data"=w128) -> ("error out"=w133:errorcluster, "Valid Selected?"=w132:bool, "Active Components"=w129:T6)  [unwired: 7 in]
            n167 = case shown="True" w132 {
              tunnel: w129 -> [_ w141]
              tunnel: w133 -> [w139 w142]
              tunnel: [w138 w143] -> w131
              tunnel: w128 -> [w137 w140]
              tunnel: [w137 w140] -> w127
              frame False {
                n168 = property class="App"() -> ("ActiveVI"=w134:string)  [unwired: 2 in, 2 out]
                n169 = String Subset(string=w134, offset (0)=1) -> (substring=w135:string)  [unwired: 1 in]
                n170 = call "Invalid Selection.vi"("error in (no error)"=w139, "Active VI"=w135) -> ("error out"=w138:errorcluster)  [unwired: 9 in]
              }
              frame True {
                n171 = call "Open Diagram.vi"("error in (no error)"=w142, "DQMH_ARG"=w141) -> ("error out"=w143:errorcluster)  [unwired: 9 in]
              }
            }
          }
          event event #0x24 {
            n172 = event-data() -> ("VIRef"=w149:refnum<vi>)  [unwired: 1 in]
            n173 = call "Save Window Position.vi"("VI Refnum"=w149) -> ()  [unwired: 10 in, 1 out]
            n174 = call-poly <vilib>:"Delacor_lib_QMH_Enqueue Message (poly).vi"("Priority Message? (F)"=TRUE, "Message"="Exit", "Message Queue in"=w144) -> ("error out"=w147:errorcluster, "Message Queue out"=w145:refnum<class "Delacor_lib_QMH_Message Queue.lvclass">)  [unwired: 7 in]
          }
          event VI Activation {
            n175 = event-data() -> ("VIAppRef"=w157:refnum<vi>, "VIName"=w160:string, "VIWindow"=w159:i32)  [unwired: 1 in]
            n176 = call "Update Active VI.vi"("VIWindow"=w159, "VIName"=w160, "Application in"=w157, "Data in"=w158) -> ("error out"=w153:errorcluster, "Changed?"=w155:bool, "Top VI"=w154:refnum<class "Standard VI Type.lvclass">, "Data out"=w161:T1)  [unwired: 4 in]
            n177 = case shown="True" w155 {
              tunnel: w151 -> [w162 w168]
              tunnel: [w163 w167] -> w156
              tunnel: w154 -> [_ w166]
              tunnel: w153 -> [w163 w165]
              tunnel: [w162 w164] -> w152
              frame False {
              }
              frame True {
                n178 = call-poly <vilib>:"Delacor_lib_QMH_Enqueue Message (poly).vi"("error in"=w165, "Message Data"=w166, "Message"="Top VI Change", "Message Queue in"=w168) -> ("error out"=w167:errorcluster, "Message Queue out"=w164:refnum<class "Delacor_lib_QMH_Message Queue.lvclass">)  [unwired: 6 in]
              }
            }
          }
          event "Peek Stack": Value Change {
            n179 = event-data() -> ("NewVal"=w172:string)  [unwired: 1 in]
            n180 = property on="Peek Stack" class="Tree (strict)"("Active Item Tag"=w172) -> ("Indent Level"=w178:i32)  [unwired: 2 in, 2 out]
            n181 = Equal To 0? "Top?"(x=w178) -> (x = 0?=w174:bool)
            n182 = Select(t="Jump to Previous" ("Message"), s=w174, f="Show Implementation" ("Message")) -> (s? t:f=w175:string)
            n183 = call-poly <vilib>:"Delacor_lib_QMH_Enqueue Message (poly).vi"("Message Data"=w172, "Message"=w175, "Message Queue in"=w170) -> ("error out"=w179:errorcluster, "Message Queue out"=w171:refnum<class "Delacor_lib_QMH_Message Queue.lvclass">)  [unwired: 7 in]
          }
          event "Previous": Value Change {
            n184 = event-data() -> ()  [unwired: 1 in, 1 out]
            n185 = call-poly <vilib>:"Delacor_lib_QMH_Enqueue Message (poly).vi"("Message"="Previous", "Message Queue in"=w181) -> ("error out"=w184:errorcluster, "Message Queue out"=w180:refnum<class "Delacor_lib_QMH_Message Queue.lvclass">)  [unwired: 8 in]
          }
          event Mouse Down? {
            n186 = event-data() -> ("Button"=w187:u16)  [unwired: 1 in, 2 out]
            n187 = Equal?(x=u16 3, y=w187) -> (x = y?=w185:bool)
            n188 = case shown="True" w185 {
              tunnel: [_ w196] -> w191
              tunnel: w189 -> [w192 w194]
              tunnel: [w192 w193] -> w188
              frame False {
              }
              frame True {
                n189 = call-poly <vilib>:"Delacor_lib_QMH_Enqueue Message (poly).vi"("Message"="Previous", "Message Queue in"=w194) -> ("error out"=w196:errorcluster, "Message Queue out"=w193:refnum<class "Delacor_lib_QMH_Message Queue.lvclass">)  [unwired: 8 in]
              }
            }
            n190 = event-data("Discard?"=w185) -> ()  [unwired: 1 in, 1 out]
          }
          event "File Open": Value Change {
            n191 = event-data() -> ()  [unwired: 1 in, 1 out]
            n192 = call-poly <vilib>:"Delacor_lib_QMH_Enqueue Message (poly).vi"("Message"="File Open", "Message Queue in"=w197) -> ("error out"=w200:errorcluster, "Message Queue out"=w198:refnum<class "Delacor_lib_QMH_Message Queue.lvclass">)  [unwired: 8 in]
          }
          event User Event {
            # "Another Module called the \"Invalid Selection\" API Method."
            n193 = event-data() -> ("Active VI"=w205:string)  [unwired: 1 in]
            n194 = Bundle(cluster=T7 {"Active VI"=""} ("Invalid Selection Argument"), "Active VI"=w205) -> (w206:T7)
            n195 = call-poly <vilib>:"Delacor_lib_QMH_Enqueue Message (poly).vi"("Message Data"=w206, "Message"="Invalid Selection", "Message Queue in"=w202) -> ("error out"=w204:errorcluster, "Message Queue out"=w203:refnum<class "Delacor_lib_QMH_Message Queue.lvclass">)  [unwired: 7 in]
          }
          event Mouse Wheel {
            n196 = event-data() -> ("Coords"=w217:T10, "Delta"=w216:i32, "PlatMods"=w215:T12)  [unwired: 1 in]
            n197 = Bundle("Coords"=w217, "Delta"=w216, "PlatMods"=w215) -> (w213:T13)  [unwired: 1 in]
            n198 = call-poly <vilib>:"Delacor_lib_QMH_Enqueue Message (poly).vi"("Message Data"=w213, "Message"="Peek Window Scroll", "Message Queue in"=w212) -> ("error out"=w210:errorcluster, "Message Queue out"=w211:refnum<class "Delacor_lib_QMH_Message Queue.lvclass">)  [unwired: 7 in]
          }
        }
        n199 = call-dynamic "Delacor_lib_QMH_Error Handler - Event Handling Loop.vi"("error in"=w47, "Message Queue in"=w38) -> ("dup error in"=w46:errorcluster)  [unwired: 8 in, 1 out]
      }
    }
    frame Error {
      # "Synchronize Caller Events.vi will inform Start Module.vi that the module has launched and will let the code calling Start Module.vi register for broadcasts and would permit the caller receive the broadcast that an error occurred at launch time."
      n200 = call-dynamic "Delacor_lib_QMH_Release Message Queue.vi"("error in"=w498, "Message Queue"=w496) -> ("error out"=w497:errorcluster)  [unwired: 9 in]
      n201 = call "Synchronize Caller Events.vi"("Singleton Module Admin in"=w499) -> ("error out"=w504:errorcluster)  [unwired: 9 in, 1 out]
      n202 = call "Module Name--constant.vi"() -> ("Module Name"=w502:string)  [unwired: 11 in]
      n203 = Format Into String(format string="An error occurred during initialization. %s is no longer running.", w502) -> (resulting string=w500:string)  [unwired: 2 in, 1 out]
      n204 = Merge Errors(w497, w504) -> (w505:errorcluster)
      n205 = call "Error Reported.vi"("Additional Information"=w500, "Error"=w505) -> ()  [unwired: 9 in, 1 out]
    }
  }
  n206 = Merge Errors(w26, w28) -> (w25:errorcluster)
  n207 = call "Close Module.vi"("error in (no error)"=w25, "Module Admin in"=w21) -> ("error out"=w27:errorcluster, "External Launch"=w14:bool, "Module Admin out"=w15:refnum<class "Delacor_lib_QMH_Module Admin.lvclass">)  [unwired: 7 in]
  n208 = Unregister For Events(event registration refnum=w20, error in=w27) -> (error out=w4:errorcluster)
  n209 = control-ref of="This VI"() -> (w2:refnum<vi>)
  n210 = call "Save Window Position.vi"("error in"=w4, "VI Refnum"=w2) -> ("error out"=w3:errorcluster)  [unwired: 9 in]
  "error out" <- w3
  n211 = case "External Launch?" shown="True" w14 {
    tunnel: w3 -> [_ w506]
    frame False {
    }
    frame True {
      n212 = case shown="Error" w506 {
        frame No Error {
          n213 = invoke on="Invoke Node" class="VI" method="FP.Close"() -> ()  [unwired: 3 in, 3 out]
        }
        frame Error {
          n214 = invoke on="Invoke Node" class="VI" method="FP.Open"("Activate"=TRUE ("Activate?")) -> ()  [unwired: 4 in, 5 out]
        }
      }
    }
  }
  n215 = local write "Module Admin"(w15) -> ()
